vi "ActiveObject_QueueQueue_Process.vi"(0 "reference in":refnum<class>, 5 "Error In":errorcluster) -> (14 "reference out":refnum<class>, 19 "Error Out":errorcluster)   [LabVIEW 2020]
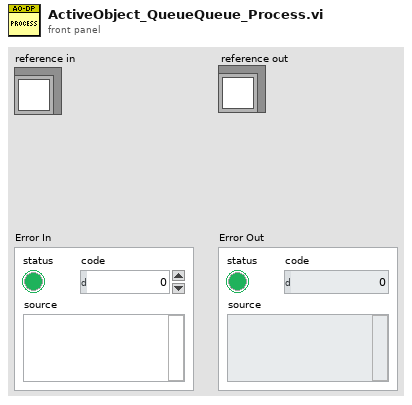
[diagram p1: front panel]
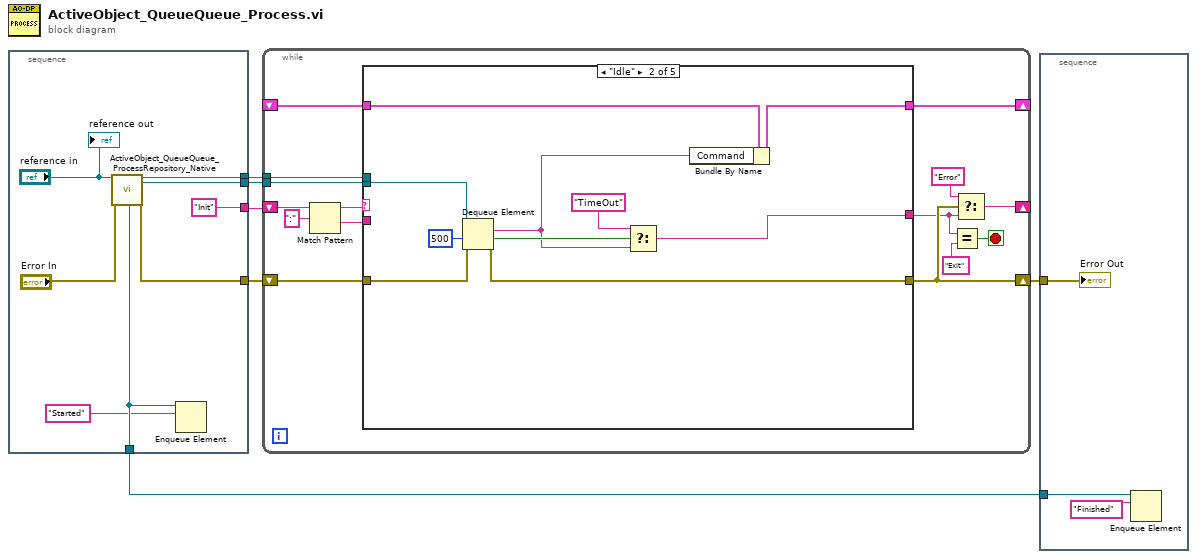
[diagram p0: block diagram]
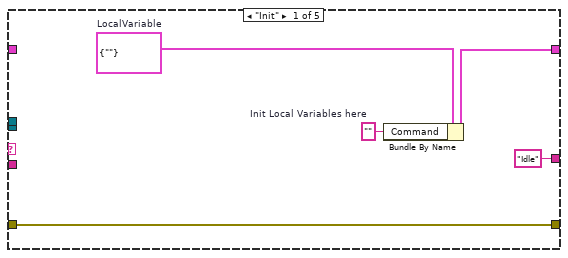
[diagram p2: hidden frame]
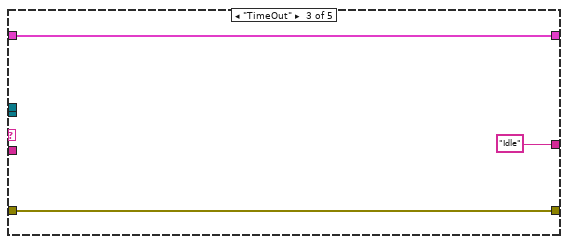
[diagram p3: hidden frame]
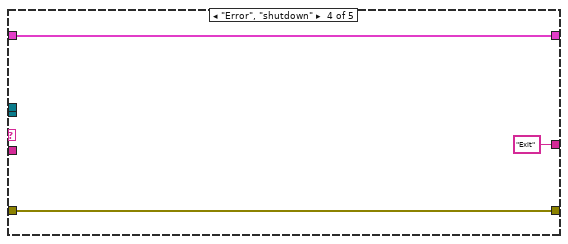
[diagram p4: hidden frame]
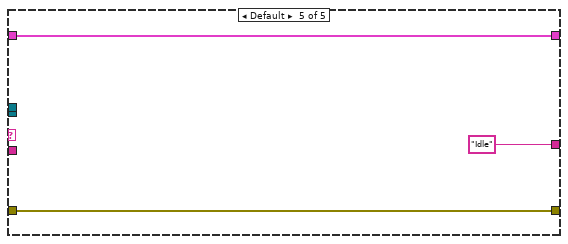
[diagram p5: hidden frame]
diagram:
  n1 = stacked-sequence {
    tunnel: [w11] -> w6
    tunnel: [w14] -> w4
    tunnel: [w10] -> w3
    tunnel: [w8] -> w2
    tunnel: ["Init"] -> w1
    frame #0 {
      n2 = call "ActiveObject_QueueQueue_ProcessRepository_Native.vi"("reference in"="reference in", "Error In"="Error In") -> ("ProcessSyncQueue"=w8:refnum<queue>, "reference out"=w14:refnum<class>, "ToProcessQueue"=w10:refnum<queue>, "Error Out"=w11:errorcluster)  [unwired: 11 in, 3 out]
      n3 = Enqueue Element(queue=w8, element="Started") -> ()  [unwired: 2 in, 3 out]
      "reference out" <- "reference in"
    }
  }
  n4 = while {
    shift-right: [w22] -> w5
    shift-left: w6 -> [w27]
    tunnel: w4 -> [w28]
    tunnel: w3 -> [w29]
    shift-right: [w20] -> _
    shift-left: w1 -> [w25]
    shift-right: [w16] -> _
    shift-left: _ -> [w15]
    stop <- w17 stop-if-true
    n5 = Match Pattern(string=w25, regular expression=":") -> (before substring=w24:string, after substring=w23:string)  [unwired: 1 in, 2 out]
    n6 = case shown="\"Idle\"" w24 {
      tunnel: w27 -> [w31 w42 w47 w50 w53]
      tunnel: [w31 w41 w47 w50 w53] -> w22
      tunnel: w29 -> [_ w43 _ _ _]
      tunnel: w28 -> [_ _ _ _ _]
      tunnel: w23 -> [_ _ _ _ _]
      tunnel: ["Idle" ("t") w38 "Idle" ("t") "Exit" ("y") "Idle" ("t")] -> w19
      tunnel: [w33 w35 w45 w48 w51] -> w16
      tunnel: w15 -> [_ w36 w45 w48 w51]
      frame "Init" {
        w32 = ""  # Init Local Variables here
        w34 = cluster{"Command":string} {"Command"=""}  # LocalVariable
        n7 = Bundle By Name(cluster=w34, "Command"=w32) -> (w33:cluster{"Command":string})
      }
      frame "Idle" {
        n8 = Dequeue Element(queue=w43, timeout in ms (-1)=500, error in (no error)=w42) -> (element=w37:string, timed out?=w40:bool, error out=w41:errorcluster)  [unwired: 1 out]
        n9 = Select(t="TimeOut", s=w40, f=w37) -> (s? t:f=w38:string)
        n10 = Bundle By Name(cluster=w36, "Command"=w37) -> (w35:cluster{"Command":string})
      }
      frame "TimeOut" {
      }
      frame "Error", "shutdown" {
      }
      frame Default {
      }
    }
    n11 = Equal?(x=w19, y="Exit") -> (x = y?=w17:bool)
    n12 = Select(t="Error", s=w22, f=w19) -> (s? t:f=w20:string)
  }
  n13 = stacked-sequence {
    tunnel: w5 -> [w56]
    tunnel: w2 -> [w55]
    frame #0 {
      n14 = Enqueue Element(queue=w55, element="Finished") -> ()  [unwired: 2 in, 3 out]
      "Error Out" <- w56
    }
  }
